vi "saveGraph.vi"(0 "reference":refnum<class "Graph.lvclass">, 1 "filePath":path, 5 "error in (no error)":errorcluster, 6 "ExportType(Normal)":T2) -> (14 "reference out":refnum<class "Graph.lvclass">, 15 "succeeded":bool, 19 "error out":errorcluster)   [LabVIEW 2020, in "Graph.lvclass"]
doc: "Save to File"
uses:
  <resource>/Framework/Providers/Open_GDS/UML/Graph_class/Graph.lvclass
  <resource>/Framework/Providers/Open_GDS/UML/Graph_class/SaveTypes.ctl
  <resource>/Framework/Providers/Open_GDS/UML/UMLEditor/UMLEditor_DiagramType.ctl
  <resource>/Framework/Providers/Open_GDS/UML/Graph_class/private/FileSaveVersionType.ctl
  <resource>/Framework/Providers/Open_GDS/UML/Graph_class/FileContent.ctl
  <resource>/Framework/Providers/Open_GDS/UML/AbstractNode_class/AbstractNode.lvclass
  <resource>/Framework/Providers/Open_GDS/UML/AbstractEdge_class/AbstractEdge.lvclass
panel:
  in  "diagramType":T1
  in  "Version(Version B)":enum16{"Oldest", "Version A", "Version B"}(ring)=enum."Version B"
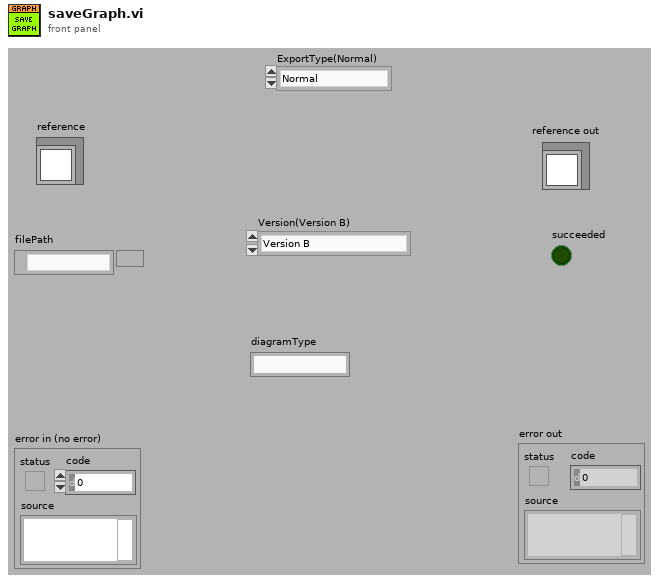
[diagram p1: front panel]
types:
  T1 = typedef "UMLEditor_DiagramType.ctl" = string
  T2 = typedef "Graph.lvclass/SaveTypes.ctl" = enum16{"Normal", "XMI"}
  T3 = enum16{"None", "Class", "Sequency", "State", "UseCase"}
  T4 = typedef "Graph.lvclass/FileContent.ctl" = cluster{"Version":string, "DiagramType":string, "DiagramData":string, "Nodes":cluster{"NodeType":string[], "ParentIndex":i32[], "ChildernIndexies":cluster{i32[]}[], "FlattenData":string[]}, "Edges":cluster{"EdgeType":string[], "StartNodeIndex":i32[], "EndNodeIndex":i32[], "FlattenData":string[]}}
  T5 = cluster{"nodeInfo":cluster{"NodeType":string[], "ParentIndex":i32[], "ChildernIndexies":cluster{i32[]}[], "FlattenData":string[]}, "edgeInfo":cluster{"EdgeType":string[], "StartNodeIndex":i32[], "EndNodeIndex":i32[], "FlattenData":string[]}, "Succeeded":bool, "DiagramData":string}
  T6 = typedef "Graph.lvclass/ObjectAttributes.ctl" = cluster{"nodes":refnum<class "AbstractNode.lvclass">[], "edges":refnum<class "AbstractEdge.lvclass">[], "nodesToBeRemoved":refnum<class "AbstractNode.lvclass">[], "edgesToBeRemoved":refnum<class "AbstractEdge.lvclass">[], "needsLayout":bool, "LayoutNodes":refnum<class "AbstractNode.lvclass">[]}
  T7 = cluster{"children":refnum<class "AbstractNode.lvclass">[]}
  T8 = cluster{"NodeType":string[], "ParentIndex":i32[], "ChildernIndexies":cluster{i32[]}[], "FlattenData":string[]}
  T9 = cluster{"EdgeType":string[], "StartNodeIndex":i32[], "EndNodeIndex":i32[], "FlattenData":string[]}
  T10 = cluster{"FileSaveVersion(Disconnected)":enum16{"A"}, "diagramType":enum16{"None", "Class", "Sequency", "State", "UseCase"}, "DiagramData":string, "nodeInfo":cluster{"NodeType":string[], "ParentIndex":i32[], "ChildernIndexies":cluster{i32[]}[], "FlattenData":string[]}, "edgeInfo":cluster{"EdgeType":string[], "StartNodeIndex":i32[], "EndNodeIndex":i32[], "FlattenData":string[]}}
  T11 = typedef "Graph.lvclass/FileSaveVersionType.ctl" = enum16{"A", "B"}
  T12 = cluster{"diagramType":enum16{"None", "Class", "Sequency", "State", "UseCase"}, "nodeInfo":cluster{"NodeType":string[], "ParentIndex":i32[], "ChildernIndexies":cluster{i32[]}[], "FlattenData":string[]}, "edgeInfo":cluster{"EdgeType":string[], "StartNodeIndex":i32[], "EndNodeIndex":i32[], "FlattenData":string[]}}
  T13 = enum16{"open", "replace", "create", "open or create", "replace or create", "replace or create with confirmation"}
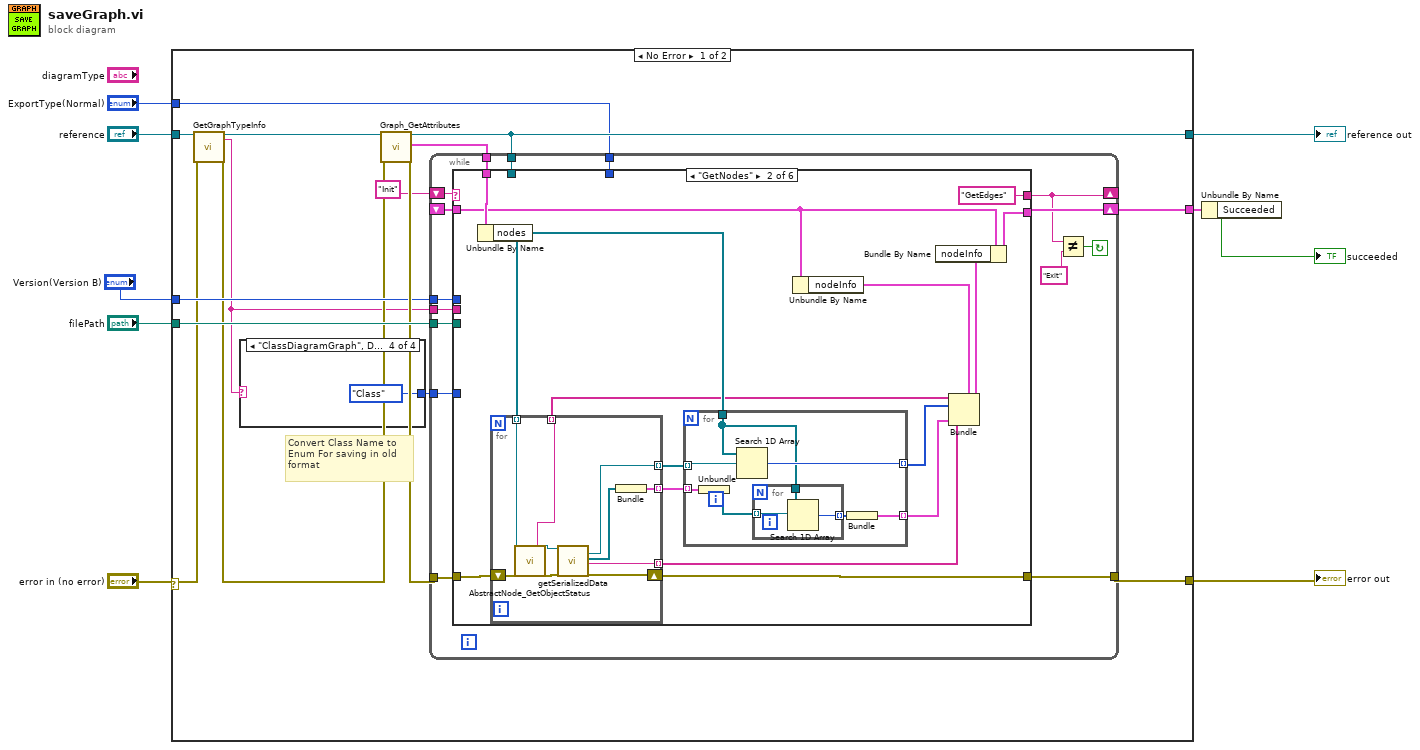
[diagram p0: block diagram]
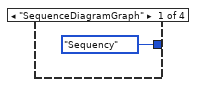
[diagram p2: hidden frame]
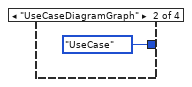
[diagram p3: hidden frame]
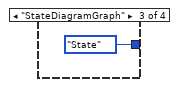
[diagram p4: hidden frame]
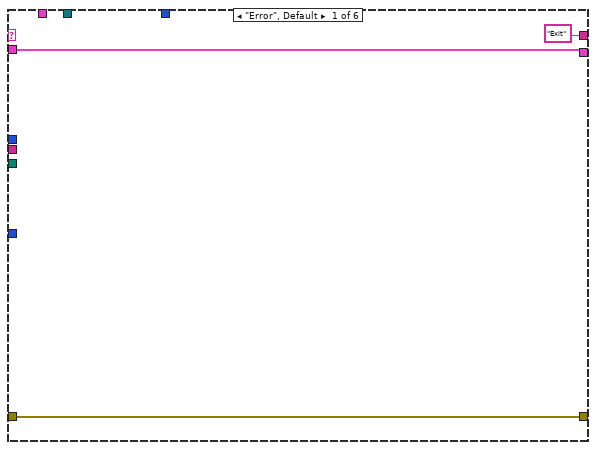
[diagram p5: hidden frame]
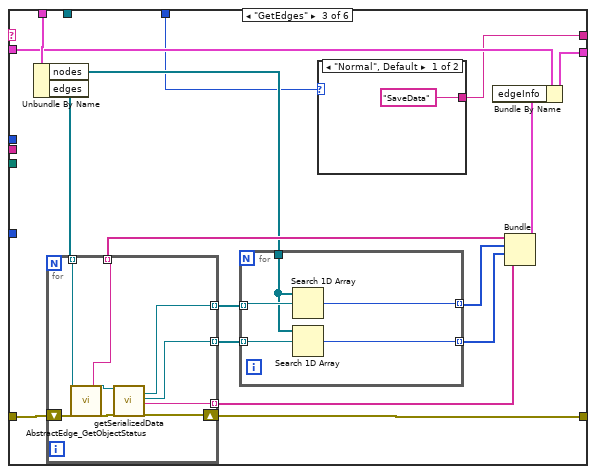
[diagram p6: hidden frame]
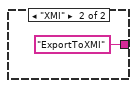
[diagram p7: hidden frame]
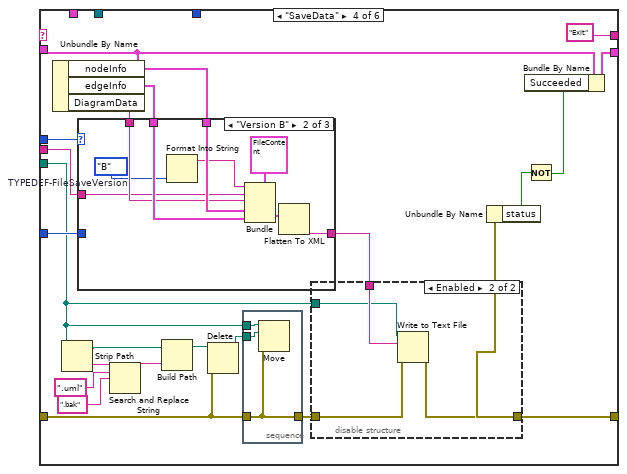
[diagram p8: hidden frame]
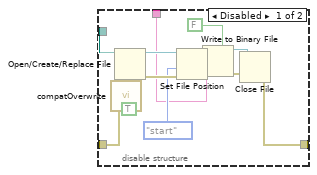
[diagram p9: hidden frame]
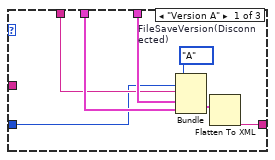
[diagram p10: hidden frame]
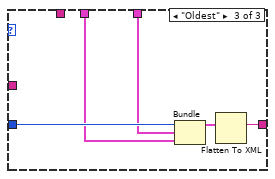
[diagram p11: hidden frame]
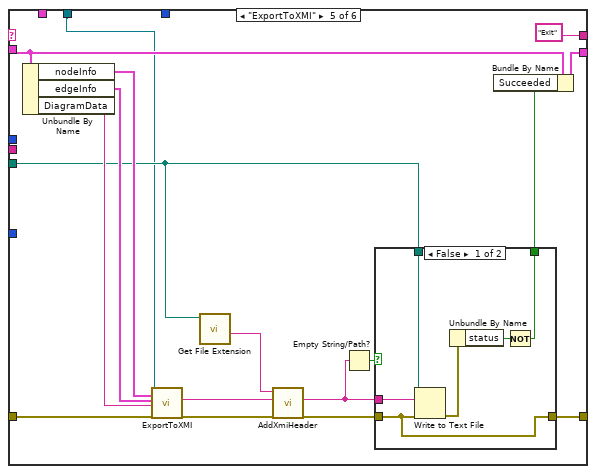
[diagram p12: hidden frame]
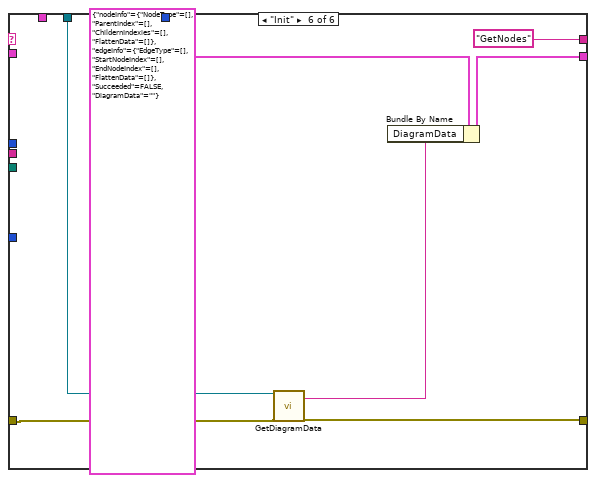
[diagram p14: hidden frame]
diagram:
  n1 = case shown="No Error" "error in (no error)" {
    selector: "error in (no error)" -> [w13 w208]
    tunnel: "reference" -> [w15 w209]
    tunnel: [w24 w208] -> w8
    tunnel: [w23 w209] -> w7
    tunnel: "filePath" -> [w22 _]
    tunnel: [w21 _] -> w4
    tunnel: "ExportType(Normal)" -> [w20 _]
    tunnel: "Version(Version B)" -> [w16 _]
    frame No Error {
      # "Convert Class Name to\nEnum For saving in old \nformat"
      n2 = call-dynamic "GetGraphTypeInfo.vi"("reference in"=w15, "error in (no error)"=w13) -> ("reference out"=w14:refnum<class "Graph.lvclass">, "GraphTypeName"=w10:string, "error out"=w12:errorcluster)  [unwired: 12 in, 3 out]
      n3 = case shown="\"ClassDiagramGraph\", Default" w10 {
        tunnel: [T3."Sequency" ("diagramType") T3."UseCase" ("diagramType") T3."State" ("diagramType") T3."Class" ("diagramType")] -> w11
        frame "SequenceDiagramGraph" {
        }
        frame "UseCaseDiagramGraph" {
        }
        frame "StateDiagramGraph" {
        }
        frame "ClassDiagramGraph", Default {
        }
      }
      n4 = call <resource>:"Graph_GetAttributes.vi"("reference in"=w14, "error in (no error)"=w12) -> ("reference out"=w23:refnum<class "Graph.lvclass">, "Data"=w17:T6, "error out"=w19:errorcluster)  [unwired: 1 in, 14 out]
      n5 = while {
        tunnel: w17 -> [w43]
        tunnel: w19 -> [w42]
        tunnel: w11 -> [w41]
        tunnel: w22 -> [w40]
        tunnel: [w39] -> w24
        shift-right: [w34] -> _
        shift-left: "Init" -> [w38]
        shift-right: [w37] -> w21
        shift-left: _ -> [w33]
        tunnel: w23 -> [w32]
        tunnel: w20 -> [w31]
        tunnel: w16 -> [w30]
        tunnel: w10 -> [w29]
        stop <- w35 continue-if-true
        n6 = case shown="\"GetNodes\"" w38 {
          tunnel: w43 -> [_ w61 w96 _ _ _]
          tunnel: w42 -> [w46 w60 w95 w118 w190 w204]
          tunnel: w41 -> [_ _ _ w133 _ _]
          tunnel: w40 -> [_ _ _ w116 w179 _]
          tunnel: [w46 w54 w91 w130 w185 w203] -> w39
          tunnel: [w44 w50 w87 w128 w192 w205] -> w37
          tunnel: ["Exit" ("y") "GetEdges" w81 "Exit" ("y") "Exit" ("y") "GetNodes"] -> w34
          tunnel: w33 -> [w44 w48 w89 w127 w191 _]
          tunnel: w32 -> [_ _ _ _ w177 w201]
          tunnel: w31 -> [_ _ w82 _ _ _]
          tunnel: w30 -> [_ _ _ w113 _ _]
          tunnel: w29 -> [_ _ _ w112 _ _]
          frame "Error", Default {
          }
          frame "GetNodes" {
            n7 = Unbundle By Name(w61) -> ("nodes"=w53:refnum<class "AbstractNode.lvclass">[])
            n8 = for {
              shift-right: [w73] -> w54
              shift-left: w60 -> [w80]
              tunnel: w53 -> [w76] mode=indexing
              tunnel: [w79] -> w59 mode=indexing
              tunnel: [w77] -> w58 mode=indexing
              tunnel: [w74] -> w55 mode=indexing
              tunnel: [w72] -> w52 mode=indexing
              n9 = call <resource>:"AbstractNode_GetObjectStatus.vi"("reference in"=w76) -> ("Class name"=w72:string, "reference out"=w75:refnum<class "AbstractNode.lvclass">)  [unwired: 1 in, 16 out]
              n10 = call-dynamic "getSerializedData.vi"("reference"=w75, "error in (no error)"=w80) -> ("parent"=w79:refnum<class "AbstractNode.lvclass">, "children"=w78:refnum<class "AbstractNode.lvclass">[], "xmlOut"=w74:string, "error out"=w73:errorcluster)  [unwired: 13 in, 1 out]
              n11 = Bundle("children"=w78) -> (w77:T7)  [unwired: 1 in]
            }
            n12 = for {
              tunnel: w59 -> [w67] mode=indexing
              tunnel: w58 -> [w68] mode=indexing
              tunnel: [w66] -> w57 mode=indexing
              tunnel: [w63] -> w56 mode=indexing
              tunnel: w53 -> [w62]
              n13 = Unbundle(w68) -> ("children"=w65:refnum<class "AbstractNode.lvclass">[])
              n14 = Search 1D Array(1D array=w62, element=w67) -> (index of element=w66:i32)  [unwired: 1 out]
              n15 = for {
                tunnel: w65 -> [w70] mode=indexing
                tunnel: w62 -> [w71]
                tunnel: [w69] -> w64 mode=indexing
                n16 = Search 1D Array(1D array=w71, element=w70) -> (index of element=w69:i32)  [unwired: 1 out]
              }
              n17 = Bundle(w64) -> (w63:cluster{i32[]})  [unwired: 1 in]
            }
            n18 = Unbundle By Name(w48) -> ("nodeInfo"=w47:T8)
            n19 = Bundle(cluster=w47, "NodeType"=w52, "ParentIndex"=w57, "ChildernIndexies"=w56, "FlattenData"=w55) -> (w51:T8)
            n20 = Bundle By Name(cluster=w48, "nodeInfo"=w51) -> (w50:T5)
          }
          frame "GetEdges" {
            n21 = Unbundle By Name(w96) -> ("nodes"=w86:refnum<class "AbstractNode.lvclass">[], "edges"=w85:refnum<class "AbstractEdge.lvclass">[])
            n22 = for {
              shift-right: [w105] -> w91
              shift-left: w95 -> [w111]
              tunnel: w85 -> [w109] mode=indexing
              tunnel: [w110] -> w94 mode=indexing
              tunnel: [w106] -> w92 mode=indexing
              tunnel: [w104] -> w90 mode=indexing
              tunnel: [w107] -> w84 mode=indexing
              n23 = call <resource>:"AbstractEdge_GetObjectStatus.vi"("reference in"=w109) -> ("Class name"=w104:string, "reference out"=w108:refnum<class "AbstractEdge.lvclass">)  [unwired: 1 in, 16 out]
              n24 = call-dynamic "getSerializedData.vi"("reference"=w108, "error in (no error)"=w111) -> ("startNode"=w110:refnum<class "AbstractNode.lvclass">, "endNode"=w107:refnum<class "AbstractNode.lvclass">, "xmlOut"=w106:string, "error out"=w105:errorcluster)  [unwired: 13 in, 1 out]
            }
            n25 = for {
              tunnel: w94 -> [w103] mode=indexing
              tunnel: [w102] -> w93 mode=indexing
              tunnel: w86 -> [w101]
              tunnel: w84 -> [w100] mode=indexing
              tunnel: [w99] -> w83 mode=indexing
              n26 = Search 1D Array(1D array=w101, element=w103) -> (index of element=w102:i32)  [unwired: 1 out]
              n27 = Search 1D Array(1D array=w101, element=w100) -> (index of element=w99:i32)  [unwired: 1 out]
            }
            n28 = case shown="\"Normal\", Default" w82 {
              tunnel: ["SaveData" "ExportToXMI"] -> w81
              frame "Normal", Default {
              }
              frame "XMI" {
              }
            }
            n29 = Bundle(w90, w93, w83, w92) -> (w88:cluster{string[], i32[], i32[], string[]})  [unwired: 1 out]
            n30 = Bundle By Name(cluster=w89, "edgeInfo"=w88) -> (w87:T5)
          }
          frame "SaveData" {
            n31 = Unbundle By Name(w127) -> ("nodeInfo"=w132:T8, "edgeInfo"=w131:T9, "DiagramData"=w115:string)
            n32 = Strip Path(path=w116) -> (stripped path=w125:path, name=w124:string)
            n33 = case shown="\"Version B\"" w113 {
              tunnel: w133 -> [w153 _ w173]
              tunnel: w132 -> [w158 w168 w172]
              tunnel: w131 -> [w157 w167 w171]
              tunnel: w115 -> [w154 w164 _]
              tunnel: [w155 w165 w169] -> w114
              tunnel: w112 -> [_ w160 _]
              frame "Version A" {
                w159 = enum16{"A"}."A"  # FileSaveVersion(Disconnected)
                n34 = Bundle("FileSaveVersion(Disconnected)"=w159, "diagramType"=w153, "DiagramData"=w154, "nodeInfo"=w158, "edgeInfo"=w157) -> (w156:T10)  [unwired: 1 out]
                n35 = Flatten To XML(6:w156) -> (2:w155:string)
              }
              frame "Version B" {
                w163 = FileSaveVersionType."B"  # TYPEDEF-FileSaveVersion
                n36 = Format Into String(w163) -> (resulting string=w162:string)  [unwired: 3 in, 1 out]
                n37 = Bundle(cluster=T4 {"Version"="", "DiagramType"="", "DiagramData"="", "Nodes"={"NodeType"=[], "ParentIndex"=[], "ChildernIndexies"=[], "FlattenData"=[]}, "Edges"={"EdgeType"=[], "StartNodeIndex"=[], "EndNodeIndex"=[], "FlattenData"=[]}}, "Version"=w162, "DiagramType"=w160, "DiagramData"=w164, "Nodes"=w168, "Edges"=w167) -> (w166:T4)
                n38 = Flatten To XML(6:w166) -> (2:w165:string)
              }
              frame "Oldest" {
                n39 = Bundle("diagramType"=w173, "nodeInfo"=w172, "edgeInfo"=w171) -> (w170:T12)  [unwired: 1 out]
                n40 = Flatten To XML(6:w170) -> (2:w169:string)
              }
            }
            n41 = Search and Replace String(input string=w124, search string=".uml", replace string=".bak" ("replace string (\"\")")) -> (result string=w121:string)  [unwired: 1 in, 7 out]
            n42 = Build Path(base path=w125, name or relative path=w121) -> (appended path=w120:path)
            n43 = Delete(path (use dialog)=w120, error in=w118) -> (deleted path=w119:path)  [unwired: 5 out]
            n44 = stacked-sequence {
              tunnel: w116 -> [w176]
              tunnel: w119 -> [w175]
              tunnel: w118 -> [w174]
              tunnel: [w174] -> w117
              frame #0 {
                n45 = Move(source path=w176, error in=w174, 10:w175) -> ()  [unwired: 5 out]
              }
            }
            n46 = disable-structure shown="Enabled" {
              disable-tunnel: [w144 w151] -> w130
              disable-tunnel: w117 -> [w141 w152]
              disable-tunnel: w116 -> [w140 w149]
              disable-tunnel: w114 -> [w139 w150]
              frame Disabled {
                n47 = call <vilib>:"compatOverwrite.vi"("overwrite (F)"=TRUE) -> ("overwrite?"=w138:T13)
                n48 = Open/Create/Replace File(file path (use dialog)=w140, error in=w141, operation (0:open)=w138) -> (refnum out=w147:refnum<file>, error out=w148:errorcluster)  [unwired: 3 in, 1 out]
                n49 = Set File Position(refnum=w147, from (0:start)=enum16{"start", "end", "current"}."start" ("pos mode (0:2)"), error in=w148) -> (refnum out=w137:refnum<file>, error out=w136:errorcluster)  [unwired: 1 out]
                n50 = Write to Binary File(file (use dialog)=w137, data=w139, error in=w136, 5:FALSE ("prepend array or string size? (T)")) -> (refnum out=w145:refnum<file>, error out=w146:errorcluster)  [unwired: 3 out]
                n51 = Close File(refnum=w145, error in=w146) -> (error out=w144:errorcluster)  [unwired: 1 out]
              }
              frame Enabled {
                n52 = Write to Text File(file (use dialog)=w149, text=w150, error in=w152) -> (error out=w151:errorcluster)  [unwired: 1 in, 2 out]
              }
            }
            n53 = Unbundle By Name(w130) -> ("status"=w129:bool)
            n54 = Not(x=w129) -> (.not. x?=w126:bool)
            n55 = Bundle By Name(cluster=w127, "Succeeded"=w126) -> (w128:T5)
          }
          frame "ExportToXMI" {
            n56 = Unbundle By Name(w191) -> ("nodeInfo"=w189:T8, "edgeInfo"=w188:T9, "DiagramData"=w187:string)
            n57 = call-dynamic "ExportToXMI.vi"("reference"=w177, "nodeInfo"=w189, "edgeInfo"=w188, "DiagramData"=w187, "error in (no error)"=w190) -> ("XMIText"=w183:string, "error out"=w182:errorcluster)  [unwired: 12 in, 1 out]
            n58 = call <vilib>:"Get File Extension.vi"("file"=w179) -> ("filename without extension"=w178:string)  [unwired: 1 in, 9 out]
            n59 = call <resource>:"AddXmiHeader.vi"("error in (no error)"=w182, "XmiContent"=w183, "DiagramName"=w178) -> ("error out"=w181:errorcluster, "XmiDocument"=w180:string)  [unwired: 7 out]
            n60 = Empty String/Path?(string/path=w180) -> (empty?=w186:bool)
            n61 = case shown="False" w186 {
              tunnel: w181 -> [w197 w200]
              tunnel: [w197 w200] -> w185
              tunnel: [w194 _] -> w184
              tunnel: w179 -> [w199 _]
              tunnel: w180 -> [w198 _]
              frame False {
                n62 = Write to Text File(file (use dialog)=w199, text=w198, error in=w197) -> (error out=w196:errorcluster)  [unwired: 3 out]
                n63 = Unbundle By Name(w196) -> ("status"=w195:bool)
                n64 = Not(x=w195) -> (.not. x?=w194:bool)
              }
              frame True {
              }
            }
            n65 = Bundle By Name(cluster=w191, "Succeeded"=w184) -> (w192:T5)
          }
          frame "Init" {
            n66 = call-dynamic "GetDiagramData.vi"("reference"=w201, "error in (no error)"=w204) -> ("DiagramData"=w202:string, "error out"=w203:errorcluster)  [unwired: 15 in, 1 out]
            n67 = Bundle By Name(cluster=T5 {"nodeInfo"={"NodeType"=[], "ParentIndex"=[], "ChildernIndexies"=[], "FlattenData"=[]}, "edgeInfo"={"EdgeType"=[], "StartNodeIndex"=[], "EndNodeIndex"=[], "FlattenData"=[]}, "Succeeded"=FALSE, "DiagramData"=""}, "DiagramData"=w202) -> (w205:T5)
          }
        }
        n68 = Not Equal?(x=w34, y="Exit") -> (x != y?=w35:bool)
      }
    }
    frame Error {
    }
  }
  "reference out" <- w7
  "error out" <- w8
  n69 = Unbundle By Name(w4) -> ("Succeeded"=→"succeeded":bool)
